vi "Initialise Serial.vi"(6 "Tag Root":string, 7 "Baud":u32=115200, 8 "error in (no error)":errorcluster, 9 "Channels":refnum<class "Abs_Value.lvclass">[](array[class]), 10 "VISA resource name":refnum<visa-resource-name>, 11 "CTI_Serial_Bus in":refnum<class "CTI_Serial_Bus.lvclass">) -> (0 "error out":errorcluster, 3 "CTI_Serial_Bus out":refnum<class "CTI_Serial_Bus.lvclass">)   [LabVIEW 2021, in "CTI_Serial_Bus.lvclass"]
uses:
  CTI_Serial_Bus.lvclass
  C:/TSA/CTI_Bus/Source/Parent/CTI_Bus.lvclass
  <vilib>/TSA/Abstract Data Classes/Abs_Types/Value/Abs_Value.lvclass
  CTI_Serial_Bus.lvclass/CTI_Serial_Bus.ctl
  Properties/Write Baud.vi
  Parent/CTI_Bus.lvclass
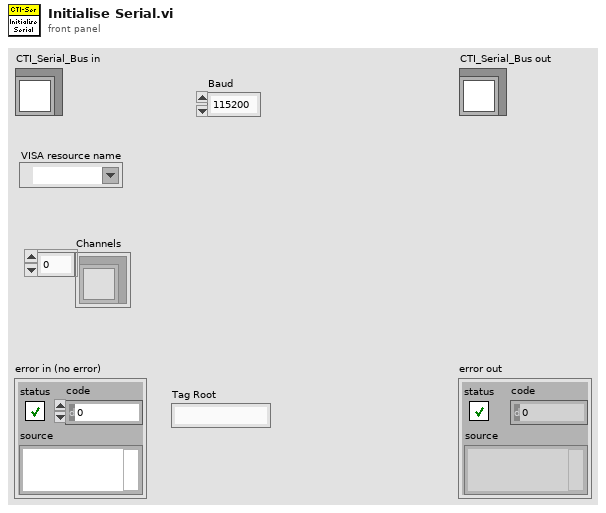
[diagram p1: front panel]
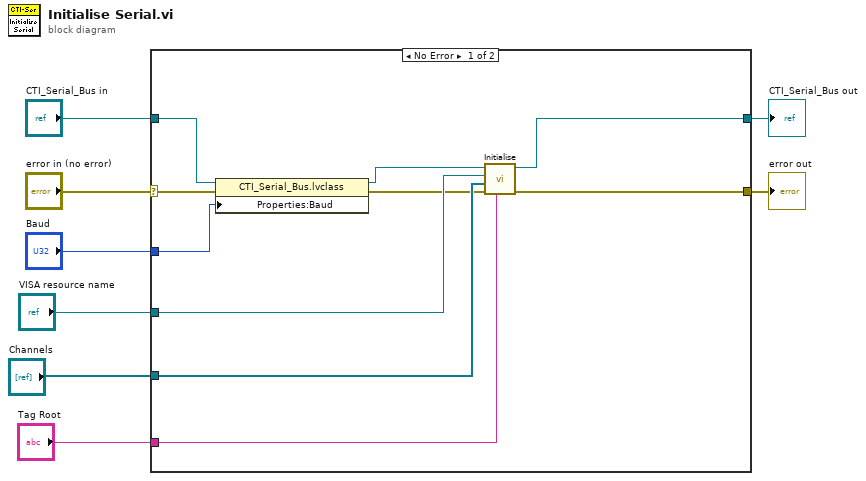
[diagram p0: block diagram]
diagram:
  n1 = case shown="No Error" "error in (no error)" {
    selector: "error in (no error)" -> [w14 w20]
    tunnel: [w18 w20] -> w7
    tunnel: [w17 w19] -> w5
    tunnel: "CTI_Serial_Bus in" -> [w12 w19]
    tunnel: "VISA resource name" -> [w16 _]
    tunnel: "Channels" -> [w15 _]
    tunnel: "Baud" -> [w10 _]
    tunnel: "Tag Root" -> [w9 _]
    frame No Error {
      n2 = property class="CTI_Serial_Bus.lvclass"(reference=w12, error in=w14, "Properties:Baud"=w10) -> (reference out=w11:refnum<class "CTI_Serial_Bus.lvclass">, error out=w13:errorcluster)
      n3 = call "Initialise.vi"("Tag Root"=w9, "error in (no error)"=w13, "Channel"=w15, "VISA resource name"=w16, "CTI_Bus in"=w11) -> ("error out"=w18:errorcluster, "CTI_Bus out"=w17:refnum<class "CTI_Serial_Bus.lvclass">)  [unwired: 5 in]
    }
    frame Error {
    }
  }
  "error out" <- w7
  "CTI_Serial_Bus out" <- w5
